vi "LOGIN_rev-1.vi"() -> ()   [LabVIEW 2021]
uses:
  Control/login_type.ctl
  Control/User_login_type.ctl
  Control/add_remove.ctl
panel:
  out "Boolean 4":bool=TRUE
  out "element 2":string
  in  "Ring - Menu 8":T1
  in  "Back Button":bool
  out "Boolean 3":bool=TRUE
  out "error in (no error) 4":errorcluster
  in  "error in (no error) 3":errorcluster
  out "Numeric":i32
  out "Enum":T2
  in  "Ring - Menu 7":T1 items=["Admin", "Operator"]
  out "element 3":string
  out "Array 2":string[](array[string])
  in  "Password 3":string
  in  "Enum":T2
  in  "error in (no error) 2":errorcluster
  in  "Remove user":bool
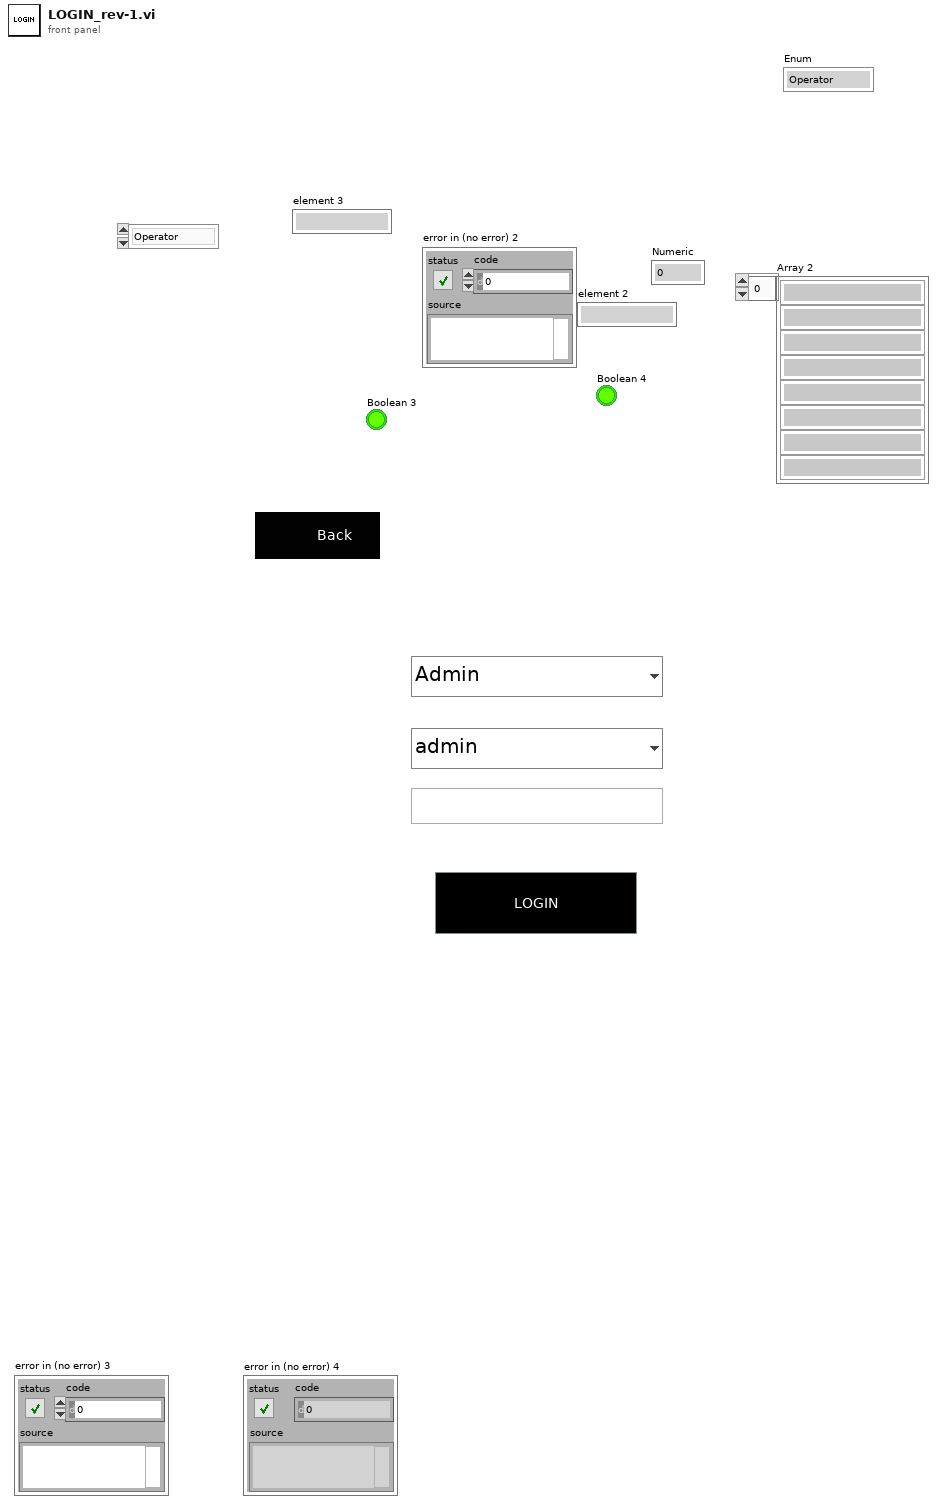
[diagram p1: front panel]
types:
  T1 = typedef "User_login_type.ctl" = u16
  T2 = typedef "login_type.ctl" = enum16{"Operator", "Admin"}
  T3 = typedef "add_remove.ctl" = enum16{"Enter", "add user", "remover user", "view user"}
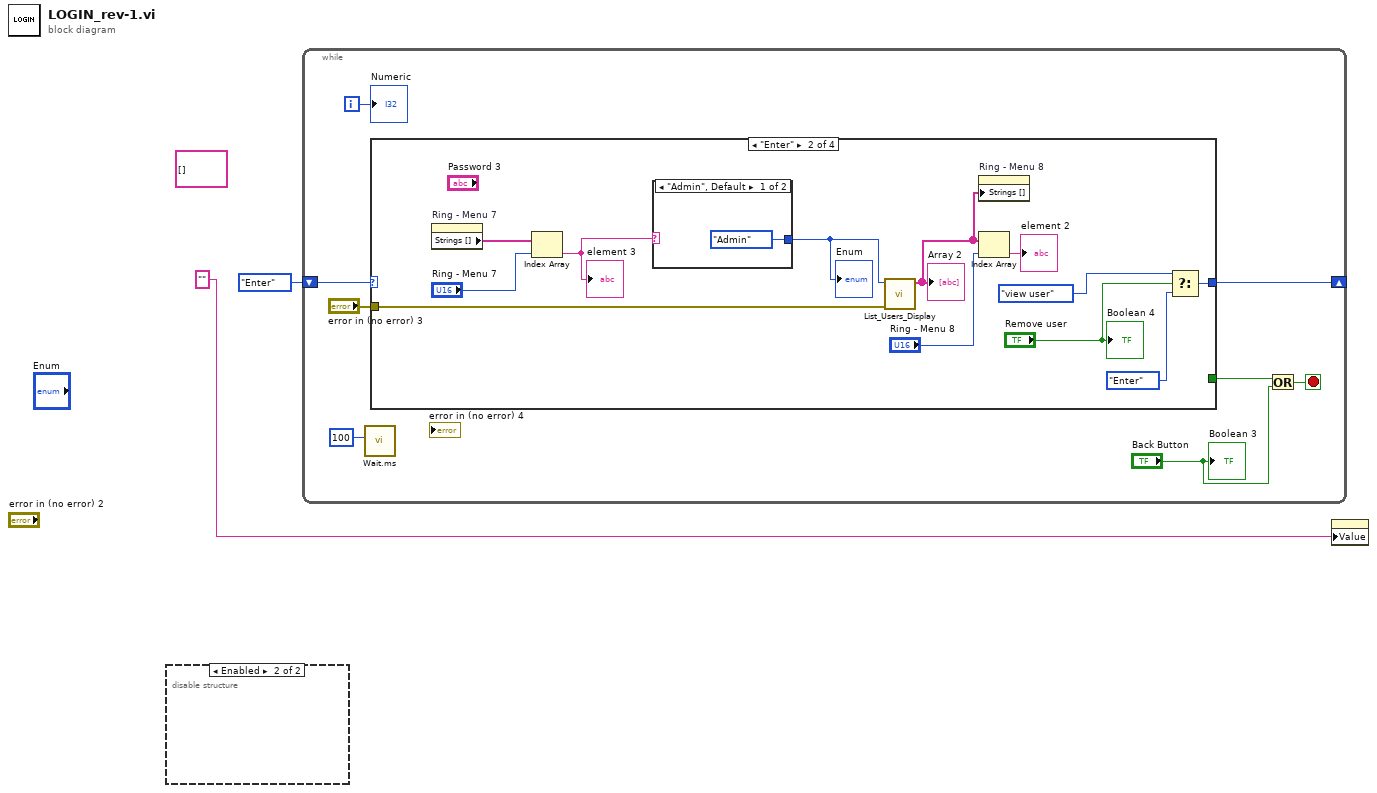
[diagram p0: block diagram]
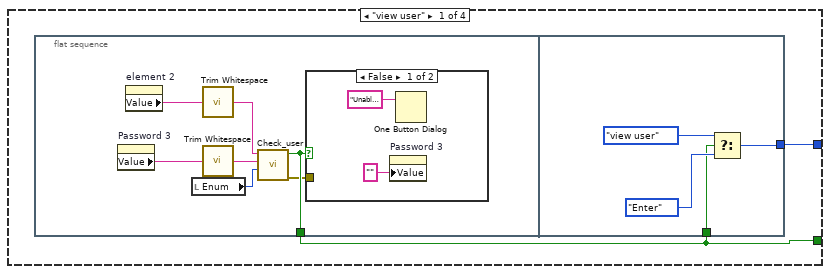
[diagram p2: hidden frame]
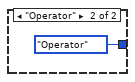
[diagram p4: hidden frame]
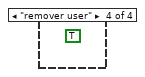
[diagram p6: hidden frame]
diagram:
  (unwired) string[][] [] ("Item Names")
  n1 = disable-structure shown="Enabled" {
    frame Disabled {
    }
    frame Enabled {
    }
  }
  n2 = while {
    shift-right: [w9] -> _
    shift-left: add_remove."Enter" -> [w10]
    i -> [w8]
    stop <- w3 stop-if-true
    n3 = call "Wait.ms.vi"("milliseconds to wait"=u32 100) -> ()  [unwired: 10 in, 1 out]
    n4 = case shown="\"Enter\"" w10 {
      tunnel: [w11 w27 _ _] -> w9
      tunnel: "error in (no error) 3" -> [_ w33 _ _]
      tunnel: [w12 _ _ _] -> w5
      frame "view user" {
        n5 = flat-sequence {
          tunnel: [w18] -> w12
          tunnel: w12 -> [w24]
          tunnel: [w22] -> w11
          frame #0 {
            n6 = property on="Password 3" class="Str"() -> ("Value"=w13:string)  [unwired: 2 in, 2 out]
            n7 = property on="element 2" class="Str"() -> ("Value"=w16:string)  [unwired: 2 in, 2 out]
            n8 = local read "Enum"() -> (w19:T2)
            n9 = call <vilib>:"Trim Whitespace.vi"("string"=w16) -> ("trimmed string"=w15:string)  [unwired: 1 in]
            n10 = call <vilib>:"Trim Whitespace.vi"("string"=w13) -> ("trimmed string"=w14:string)  [unwired: 1 in]
            n11 = call "Check_user.vi"("Enum"=w19, "Password"=w14, "Name"=w15) -> ("error out"=w17:errorcluster, "Result"=w18:bool)  [unwired: 7 in]
            n12 = case shown="False" w18 {
              tunnel: w17 -> [_ _]
              frame False {
                n13 = property on="Password 3" class="Str"("Value"="" ("Password 3")) -> ()  [unwired: 2 in, 2 out]
                n14 = One Button Dialog(message="Unable to login Check ID and password") -> ()  [unwired: 1 in, 1 out]
              }
              frame True {
              }
            }
          }
          frame #1 {
            n15 = Select(t=add_remove."view user", s=w24, f=add_remove."Enter") -> (s? t:f=w22:T3)
          }
        }
      }
      frame "Enter" {
        n16 = property on="Ring - Menu 7" class="Ring (strict)"() -> ("Strings []"=w37:string[])  [unwired: 2 in, 2 out]
        n17 = Index Array(array=w37, index="Ring - Menu 7") -> (element=w35:string)
        "element 3" <- w35
        n18 = case shown="\"Admin\", Default" w35 {
          tunnel: [login_type."Admin" login_type."Operator"] -> w34
          frame "Admin", Default {
          }
          frame "Operator" {
          }
        }
        "Enum" <- w34
        n19 = call "List_Users_Display.vi"("error in (no error)"=w33, "Enum"=w34) -> ("Array"=w32:string[])  [unwired: 8 in, 1 out]
        "Array 2" <- w32
        n20 = property on="Ring - Menu 8" class="Ring (strict)"("Strings []"=w32) -> ()  [unwired: 2 in, 2 out]
        n21 = Index Array(array=w32, index="Ring - Menu 8") -> (element=→"element 2":string)
        n22 = Select(t=add_remove."view user", s="Remove user", f=add_remove."Enter") -> (s? t:f=w27:T3)
        "Boolean 4" <- "Remove user"
      }
      frame "add user" {
      }
      frame "remover user" {
        (unwired) TRUE
      }
    }
    n23 = Or(x=w5, y="Back Button") -> (x .or. y?=w3:bool)
    "Numeric" <- w8
    "Boolean 3" <- "Back Button"
  }
  n24 = property on="Password 3" class="Str"("Value"="" ("Name 3")) -> ()  [unwired: 2 in, 2 out]
